vi "SwerveDrivePoseEst_ResetPosition.vi"(8 "ModulePositions":T1[](array[typedef]) {"Angle"."SIN" format="%13.4f"; "Angle"."COS" format="%13.4f"; "Angle"."VALUE" format="%13.4f"}, 9 "Gyro":T2={"VALUE"=0.0, "COS"=1.0, "SIN"=0.0} {"SIN" format="%13.4f"; "COS" format="%13.4f"; "VALUE" format="%13.4f"}, 10 "Pose":T12={"TRANSLATION"={"X"=0.0, "Y"=0.0}, "ROTATION"={"VALUE"=0.0, "COS"=1.0, "SIN"=0.0}} {"ROTATION"."SIN" format="%13.4f"; "ROTATION"."COS" format="%13.4f"; "ROTATION"."VALUE" format="%13.4f"; "TRANSLATION"."Y" format="%14.3f"; "TRANSLATION"."X" format="%14.3f"}, 11 "in SwerveDrivePoseEstimate":T3={"M_VisionContR"=[], "m_nominal_dT"=0.0, "m_PrevTime_Sec"=0.0, "m_GyroOffset"={"VALUE"=0.0, "COS"=1.0, "SIN"=0.0}, "m_PrevAngle"={"VALUE"=0.0, "COS"=1.0, "SIN"=0.0}, "m_Observer"={"m_P"=[], "m_xHat"=[], "States"=0, "Outputs"=0, "m_ContR"=[], "m_ContQ"=[], "m_SigmasF"=[], "m_dT_Sec"=0.0, "MERWE_SCALED_SIGMA_PTS"={"m_Wm"=[], "States"=0, "Alpha"=0.0, "m_Wc"=[], "Kappa"=0}, "meanFuncX"=refnum, "meanFuncY"=refnum, "residualFuncX"=refnum, "residualFuncY"=refnum, "addFuncX"=refnum, "addFuncXExtra"=variant, "residualFuncYExtra"=variant, "residualFuncXExtra"=variant, "MeanFuncYExtra"=variant, "MeanFuncXExtra"=variant, "Inputs"=0}, "m_kinematics"={"NumModules"=0, "InverseKinematics"=[], "ForwardKinematics"=[], "Modules"=[], "PrevCoR"={"X"=0.0, "Y"=0.0}, "SavedModuleStates"=[]}, "Pose_Buffer"={"TimeStamps"=[], "Pose"=[], "Min_TimeStamp"=0.0, "Max_TimeStamp"=0.0, "ItemCount"=0, "MaxBufferTime"=0.0}, "States"=0, "Inputs"=0, "Outputs"=0} {"Pose_Buffer"."Pose"."ROTATION"."SIN" format="%13.4f"; "Pose_Buffer"."Pose"."ROTATION"."COS" format="%13.4f"; "Pose_Buffer"."Pose"."ROTATION"."VALUE" format="%13.4f"; "Pose_Buffer"."Pose"."TRANSLATION"."Y" format="%14.3f"; "Pose_Buffer"."Pose"."TRANSLATION"."X" format="%14.3f"; "m_kinematics"."SavedModuleStates"."Angle"."SIN" format="%13.4f"; "m_kinematics"."SavedModuleStates"."Angle"."COS" format="%13.4f"; "m_kinematics"."SavedModuleStates"."Angle"."VALUE" format="%13.4f"; "m_kinematics"."PrevCoR"."Y" format="%14.3f"; "m_kinematics"."PrevCoR"."X" format="%14.3f"; "m_kinematics"."Modules"."Y" format="%14.3f"; "m_kinematics"."Modules"."X" format="%14.3f"; "m_PrevAngle"."SIN" format="%13.4f"; "m_PrevAngle"."COS" format="%13.4f"; "m_PrevAngle"."VALUE" format="%13.4f"; "m_GyroOffset"."SIN" format="%13.4f"; "m_GyroOffset"."COS" format="%13.4f"; "m_GyroOffset"."VALUE" format="%13.4f"}) -> (0 "Error":bool, 3 "Out SwerveDrivePoseEstimate":T3={"M_VisionContR"=[], "m_nominal_dT"=0.0, "m_PrevTime_Sec"=0.0, "m_GyroOffset"={"VALUE"=0.0, "COS"=1.0, "SIN"=0.0}, "m_PrevAngle"={"VALUE"=0.0, "COS"=1.0, "SIN"=0.0}, "m_Observer"={"m_P"=[], "m_xHat"=[], "States"=0, "Outputs"=0, "m_ContR"=[], "m_ContQ"=[], "m_SigmasF"=[], "m_dT_Sec"=0.0, "MERWE_SCALED_SIGMA_PTS"={"m_Wm"=[], "States"=0, "Alpha"=0.0, "m_Wc"=[], "Kappa"=0}, "meanFuncX"=refnum, "meanFuncY"=refnum, "residualFuncX"=refnum, "residualFuncY"=refnum, "addFuncX"=refnum, "addFuncXExtra"=variant, "residualFuncYExtra"=variant, "residualFuncXExtra"=variant, "MeanFuncYExtra"=variant, "MeanFuncXExtra"=variant, "Inputs"=0}, "m_kinematics"={"NumModules"=0, "InverseKinematics"=[], "ForwardKinematics"=[], "Modules"=[], "PrevCoR"={"X"=0.0, "Y"=0.0}, "SavedModuleStates"=[]}, "Pose_Buffer"={"TimeStamps"=[], "Pose"=[], "Min_TimeStamp"=0.0, "Max_TimeStamp"=0.0, "ItemCount"=0, "MaxBufferTime"=0.0}, "States"=0, "Inputs"=0, "Outputs"=0} {"Pose_Buffer"."Pose"."ROTATION"."SIN" format="%13.4f"; "Pose_Buffer"."Pose"."ROTATION"."COS" format="%13.4f"; "Pose_Buffer"."Pose"."ROTATION"."VALUE" format="%13.4f"; "Pose_Buffer"."Pose"."TRANSLATION"."Y" format="%14.3f"; "Pose_Buffer"."Pose"."TRANSLATION"."X" format="%14.3f"; "m_kinematics"."SavedModuleStates"."Angle"."SIN" format="%13.4f"; "m_kinematics"."SavedModuleStates"."Angle"."COS" format="%13.4f"; "m_kinematics"."SavedModuleStates"."Angle"."VALUE" format="%13.4f"; "m_kinematics"."PrevCoR"."Y" format="%14.3f"; "m_kinematics"."PrevCoR"."X" format="%14.3f"; "m_kinematics"."Modules"."Y" format="%14.3f"; "m_kinematics"."Modules"."X" format="%14.3f"; "m_PrevAngle"."SIN" format="%13.4f"; "m_PrevAngle"."COS" format="%13.4f"; "m_PrevAngle"."VALUE" format="%13.4f"; "m_GyroOffset"."SIN" format="%13.4f"; "m_GyroOffset"."COS" format="%13.4f"; "m_GyroOffset"."VALUE" format="%13.4f"})   [LabVIEW 2019, in "Trajectory_Library.lvlib"]
doc: "This set of functions is deprecated. Suggest using the new Swerve Drive Pose Est 2 instead.\n\nResets the robot's position on the field.\n \n(NOTE -- For LabVIEW version, this may not be needed.) You NEED to reset your encoders (to zero) when calling this method.\n \nThe gyroscope angle does not need to be reset in the user's robot code. The library automatically takes care of offsetting the gyro angle.\n \nInputs:\n - SwervePoseEst -- Data cluster containing SwervePoseEst data\n - poseMeters -- The position on the field that your robot is at.\n - gyroAngle -- The angle reported by the gyroscope.\n - modulePositions -- The current distance measurements and rotations of the swerve modules.\n\nOutputs:\n - outSwevePoseEst -- Updated data cluster"
uses:
  Trajectory_Library.lvlib
  TypeDef/SWERVE_DRIVE_POSE_EST.ctl
  <vilib>/Analysis/Matrix/Datatypes/RealMatrix.ctl
  TypeDef/ROTATION2D.ctl
  TypeDef/UNSCENTED_KALMAN_FILTER.ctl
  TypeDef/MERWE_SCALED_SIGMA_PTS.ctl
  TypeDef/CALLBACK_FUNC_TYPE.ctl
  TypeDef/SWERVE_DRIVE_KINEMATICS.ctl
  TypeDef/TRANSLATION2D.ctl
  TypeDef/SWERVE_DRIVE_MODULE_STATE.ctl
  TypeDef/TIME_INTERPOLATABLE_POSE2D.ctl
  TypeDef/POSE2D.ctl
  TypeDef/SWERVE_DRIVE_MODULE_POSITION.ctl
  VecBuilder_3x1Fill.vi
  Pose2d_getXYAngle.vi
  MatBuilder_Create.vi
  Rotation2d_UnaryMinus.vi
  Rotation2d_RotateBy.vi
  Rotation2d_CreateAngle.vi
  Rotation2d_CreateXY.vi
  Util_CalcDist.vi
  <vilib>/Analysis/Matrix/NI_Matrix.lvlib
panel:
  # "<3, 3>"
  # "State Estimate <Statess,1>"
  # "<States, States>"
  # "<States, ?>"
  # "<Statess,  States>"
  # "<Outputs, Outputs>"
  # "<?, 1>"
  # "<?, 1>"
  # "<3, 3>"
  # "State Estimate <Statess,1>"
  # "<States, States>"
  # "<States, ?>"
  # "<Statess,  States>"
  # "<Outputs, Outputs>"
  # "<?, 1>"
  # "<?, 1>"
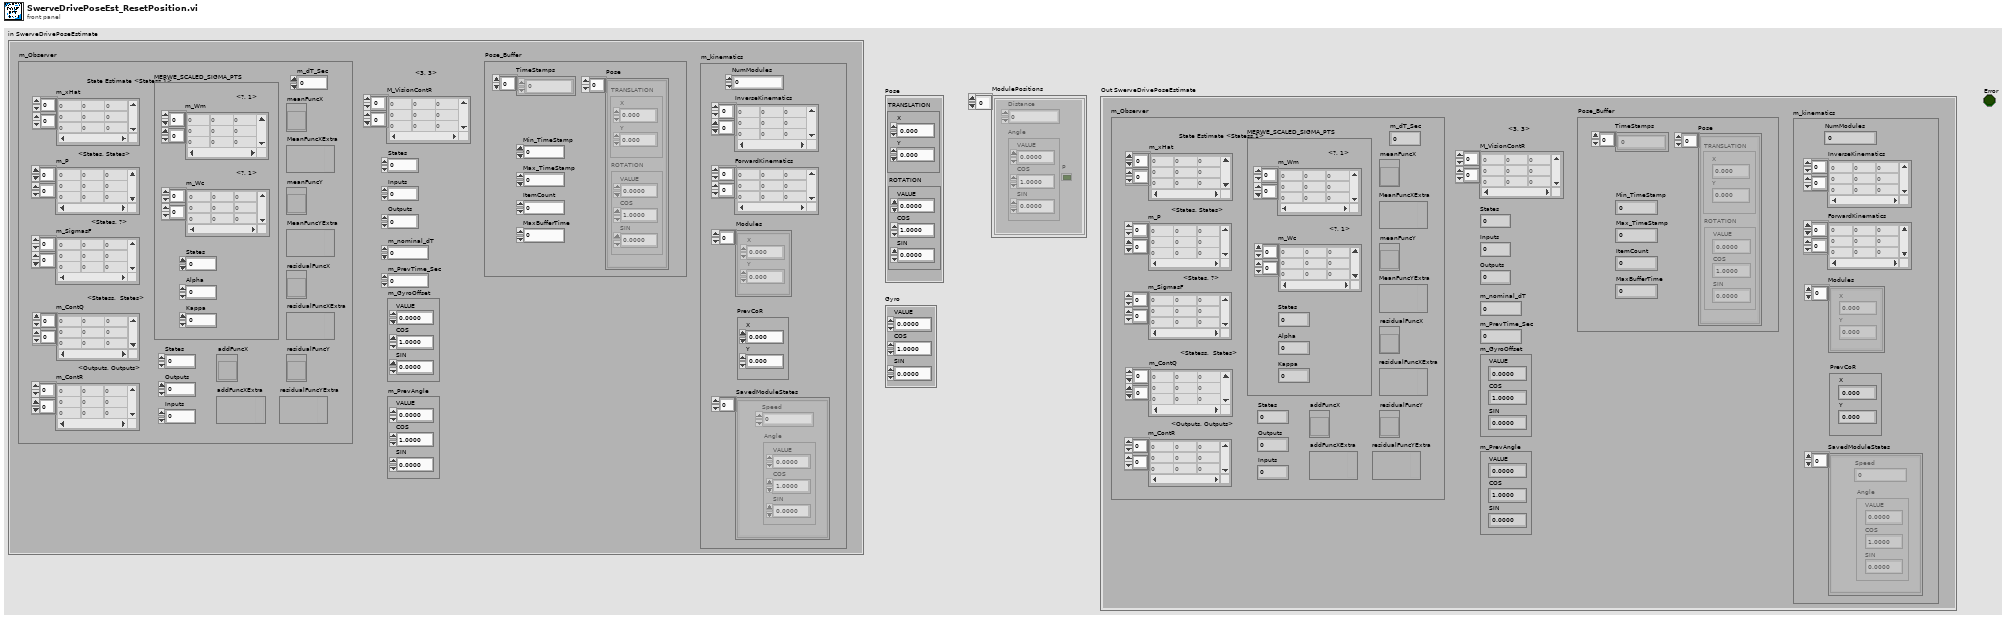
[diagram p1: front panel]
types:
  T1 = typedef "Trajectory_Library.lvlib/SWERVE_DRIVE_MODULE_POSITION.ctl" = cluster{"Distance":dbl, "Angle":T2, "P":bool}
  T2 = typedef "Trajectory_Library.lvlib/ROTATION2D.ctl" = cluster{"VALUE":dbl, "COS":dbl, "SIN":dbl}
  T3 = typedef "Trajectory_Library.lvlib/SWERVE_DRIVE_POSE_EST.ctl" = cluster{"M_VisionContR":T4, "m_nominal_dT":dbl, "m_PrevTime_Sec":dbl, "m_GyroOffset":T2, "m_PrevAngle":T2, "m_Observer":T5, "m_kinematics":T8, "Pose_Buffer":T11, "States":i32, "Inputs":i32, "Outputs":i32}
  T4 = typedef "NI_Matrix.lvlib/RealMatrix.ctl" = dbl[][]
  T5 = typedef "Trajectory_Library.lvlib/UNSCENTED_KALMAN_FILTER.ctl" = cluster{"m_P":T4, "m_xHat":T4, "States":i32, "Outputs":i32, "m_ContR":T4, "m_ContQ":T4, "m_SigmasF":T4, "m_dT_Sec":dbl, "MERWE_SCALED_SIGMA_PTS":T6, "meanFuncX":T7, "meanFuncY":T7, "residualFuncX":T7, "residualFuncY":T7, "addFuncX":T7, "addFuncXExtra":variant, "residualFuncYExtra":variant, "residualFuncXExtra":variant, "MeanFuncYExtra":variant, "MeanFuncXExtra":variant, "Inputs":i32}
  T6 = typedef "Trajectory_Library.lvlib/MERWE_SCALED_SIGMA_PTS.ctl" = cluster{"m_Wm":T4, "States":i32, "Alpha":dbl, "m_Wc":T4, "Kappa":i32}
  T7 = typedef "Trajectory_Library.lvlib/CALLBACK_FUNC_TYPE.ctl" = refnum<vi>
  T8 = typedef "Trajectory_Library.lvlib/SWERVE_DRIVE_KINEMATICS.ctl" = cluster{"NumModules":i32, "InverseKinematics":T4, "ForwardKinematics":T4, "Modules":T9[], "PrevCoR":T9, "SavedModuleStates":T10[]}
  T9 = typedef "Trajectory_Library.lvlib/TRANSLATION2D.ctl" = cluster{"X":dbl, "Y":dbl}
  T10 = typedef "Trajectory_Library.lvlib/SWERVE_DRIVE_MODULE_STATE.ctl" = cluster{"Speed":dbl, "Angle":T2}
  T11 = typedef "Trajectory_Library.lvlib/TIME_INTERPOLATABLE_POSE2D.ctl" = cluster{"TimeStamps":dbl[], "Pose":T12[], "Min_TimeStamp":dbl, "Max_TimeStamp":dbl, "ItemCount":i32, "MaxBufferTime":dbl}
  T12 = typedef "Trajectory_Library.lvlib/POSE2D.ctl" = cluster{"TRANSLATION":T9, "ROTATION":T2}
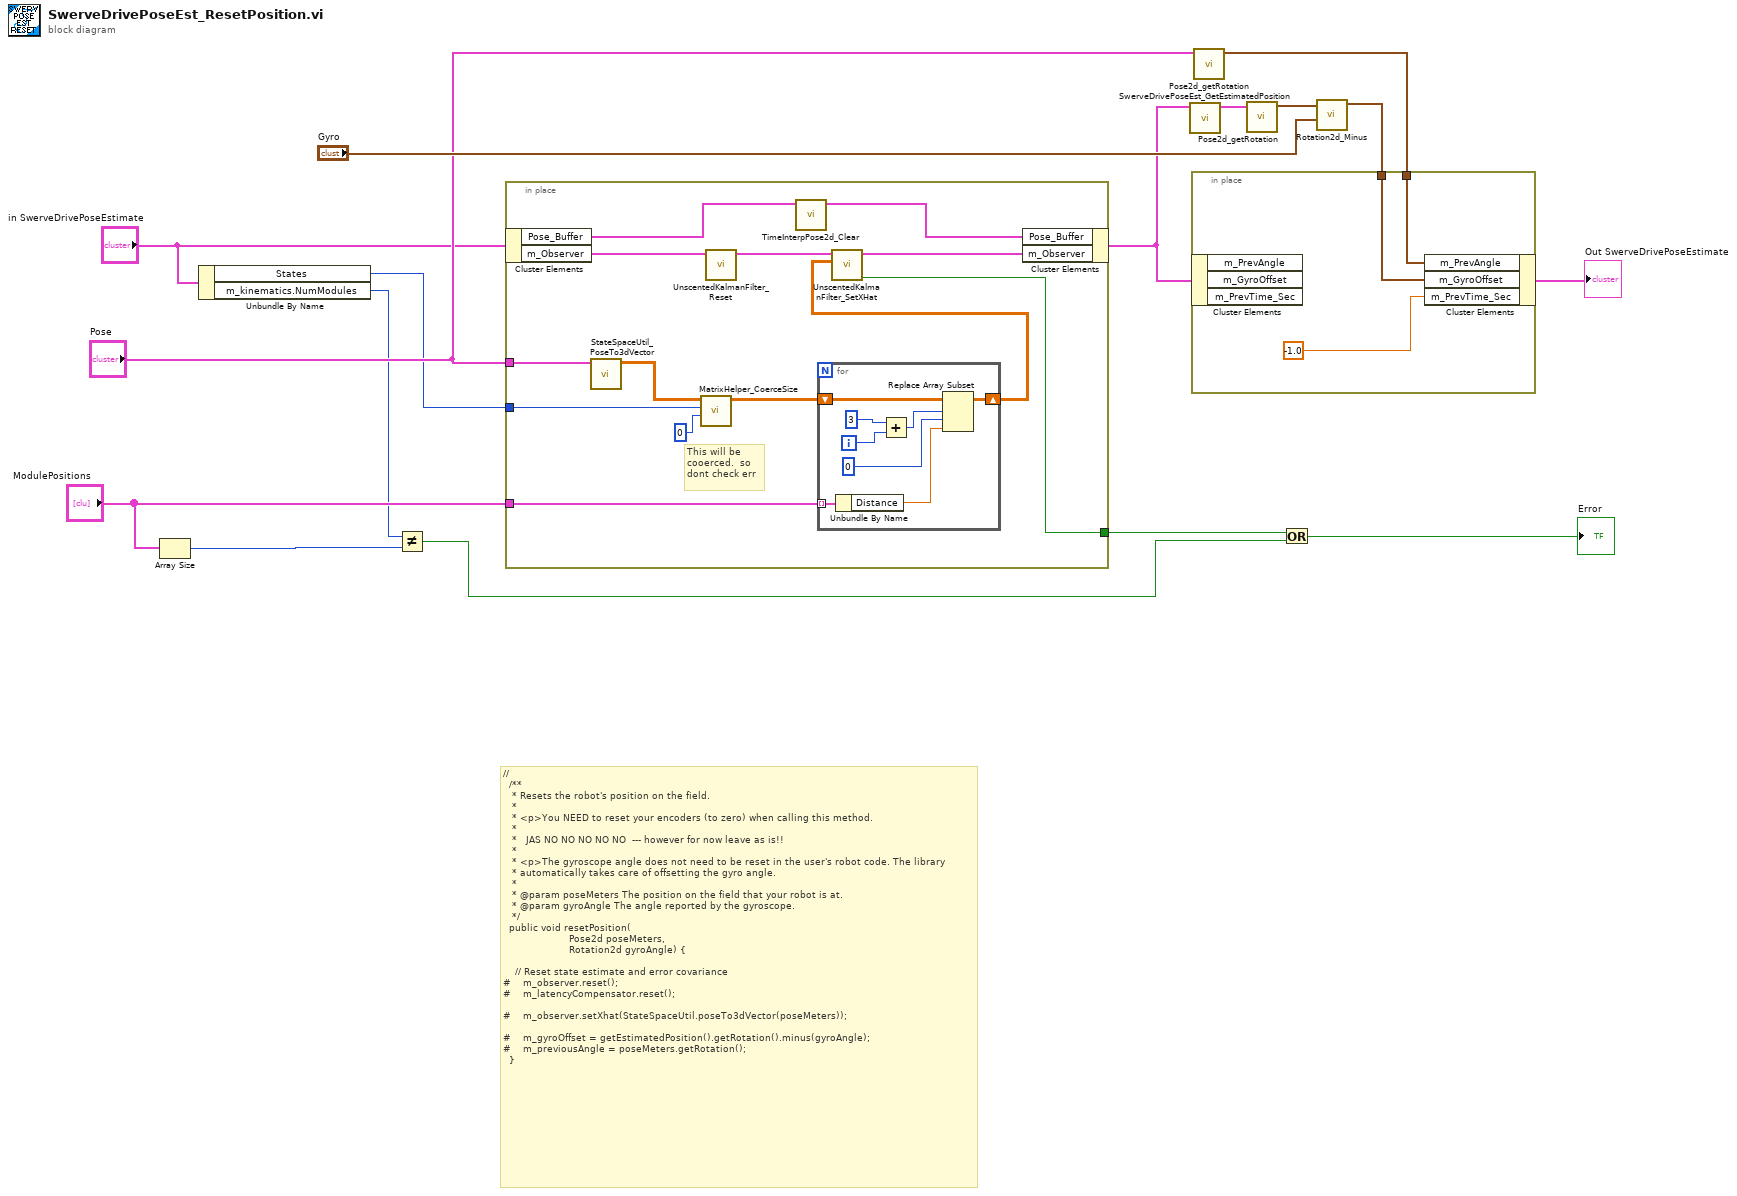
[diagram p0: block diagram]
diagram:
  # "// \n  /**\n   * Resets the robot's position on the field.\n   *\n   * <p>You NEED to reset your encoders (to zero) when calling this method.  \n   *  \n   *   JAS NO NO NO NO NO  --- however for now leave as is!!\n   *\n   * <p>The gyroscope angle does not need to be reset in the user's robot code. The library\n   * automatically takes care of offsetting the gyro angle.\n   *\n   * @param poseMeters The position on the field that your robot is at.\n   * @param gyroAngle The angle reported by the gyroscope.\n   */\n  public void resetPosition(\n                      Pose2d poseMeters, \n                      Rotation2d gyroAngle) {\n\n    // Reset state estimate and error covariance\n#    m_observer.reset();\n#    m_latencyCompensator.reset();\n\n#    m_observer.setXhat(StateSpaceUtil.poseTo3dVector(poseMeters));\n\n#    m_gyroOffset = getEstimatedPosition().getRotation().minus(gyroAngle);\n#    m_previousAngle = poseMeters.getRotation();\n  }"
  n1 = Array Size(array="ModulePositions") -> (size(s)=w4:i32)
  n2 = Unbundle By Name("in SwerveDrivePoseEstimate") -> ("States"=w7:i32, "m_kinematics.NumModules"=w5:i32)
  n3 = Not Equal?(x=w5, y=w4) -> (x != y?=w2:bool)
  n4 = in-place {
    in-place-border: "Pose" -> [w26]
    in-place-border: w7 -> [w20]
    in-place-border: "ModulePositions" -> [w19]
    in-place-border: [w17] -> w3
    # "This will be\ncooerced.  so\ndont check err"
    n5 = in-place-cluster #1("in SwerveDrivePoseEstimate") -> ("Pose_Buffer"=w25:T11, "m_Observer"=w28:T5)
    n6 = call "StateSpaceUtil_PoseTo3dVector.vi"("Pose"=w26) -> ("Pose Vector"=w21:T4)  [unwired: 10 in]
    n7 = call "MatrixHelper_CoerceSize.vi"("Columns"=0, "Rows"=w20, "input matrix"=w21) -> ("output matrix"=w23:T4)  [unwired: 7 in, 1 out]
    n8 = call "UnscentedKalmanFilter_Reset.vi"("in UnscentedKalmanFiilter"=w28) -> ("out UnscentedKalmanFiilter"=w29:T5)  [unwired: 10 in]
    n9 = call "TimeInterpPose2d_Clear.vi"("in TimeInterpPose"=w25) -> ("out TimeInterpPose"=w24:T11)  [unwired: 10 in]
    n10 = for {
      tunnel: w19 -> [w37] mode=indexing
      shift-right: [w30] -> w18
      shift-left: w23 -> [w34]
      i -> [w35]
      n11 = Unbundle By Name(w37) -> ("Distance"=w31:dbl)
      n12 = Add(x=3 ("States"), y=w35) -> (x+y=w33:i32)
      n13 = Replace Array Subset(array=w34, new element=w31, index (row)=w33, index (col)=0 ("disabled index (col)")) -> (w30:T4)
    }
    n14 = call "UnscentedKalmanFilter_SetXHat.vi"("xHat"=w18, "in UnscentedKalmanFiilter"=w29) -> ("SizeCoerced"=w17:bool, "out UnscentedKalmanFiilter"=w27:T5)  [unwired: 8 in]
    n15 = in-place-cluster #1("Pose_Buffer"=w24, "m_Observer"=w27) -> (w13:T3)
  }
  n16 = call "SwerveDrivePoseEst_GetEstimatedPosition.vi"("in SwerveDrivePoseEstimate"=w13) -> ("Estimated Pose"=w16:T12)  [unwired: 10 in]
  n17 = call "Pose2d_getRotation.vi"("in POSE"="Pose") -> ("out ROTATION"=w10:T2)  [unwired: 10 in]
  n18 = call "Pose2d_getRotation.vi"("in POSE"=w16) -> ("out ROTATION"=w14:T2)  [unwired: 10 in]
  n19 = Or(x=w3, y=w2) -> (x .or. y?=→"Error":bool)
  n20 = call "Rotation2d_Minus.vi"("other ROTATION"="Gyro", "in ROTATION"=w14) -> ("out ROTATION"=w12:T2)  [unwired: 9 in]
  n21 = in-place {
    in-place-border: w12 -> [w39]
    in-place-border: w10 -> [w38]
    n22 = in-place-cluster #2(w13) -> ()  [unwired: 3 out]
    n23 = in-place-cluster #2("m_PrevAngle"=w38, "m_GyroOffset"=w39, "m_PrevTime_Sec"=-1.0) -> (→"Out SwerveDrivePoseEstimate":T3)
  }
